vi "order-spectrum-flexlogger-hold-test.vi"(8 "error in (no error)":errorcluster) -> (0 "error out":errorcluster, 1 "Plot Waveform Count":i32[](array[numeric]), 2 "Plot Values":dbl[][][](array[numeric]), 3 "Log Values":dbl[][](array[numeric]), 4 "Log Waveform Count":i32[](array[numeric]))   [LabVIEW 2026]
doc: "Hold/reset unit test for OrderSpectrumToFlexLogger.vi: calls it 5 times with (0) reset + spectrum A, (1) empty magnitude, (2) empty array, (3) spectrum B, (4) reset + empty array. Returns numeric arrays only."
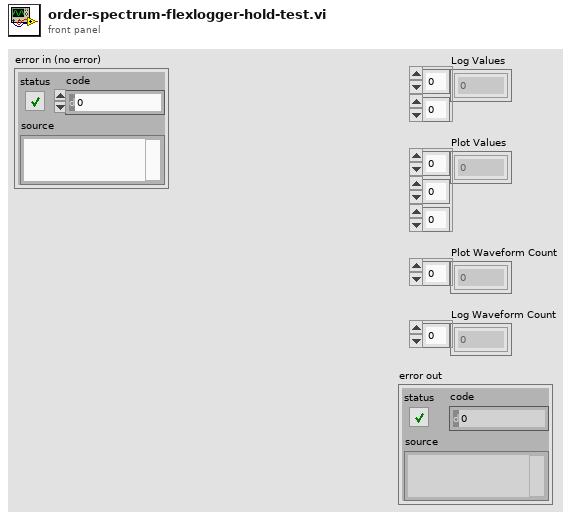
[diagram p1: front panel]
types:
  T1 = cluster{"channels":i32, "plot points per block":i32, "plot in dB? (F)":bool, "window ENBW (bins)":dbl}
  T2 = cluster{"spectra":cluster{"order 0":dbl, "delta order":dbl, "magnitude":dbl[]}[], "reset":bool}[]
  T3 = cluster{"order 0":dbl, "delta order":dbl, "magnitude":dbl[]}[]
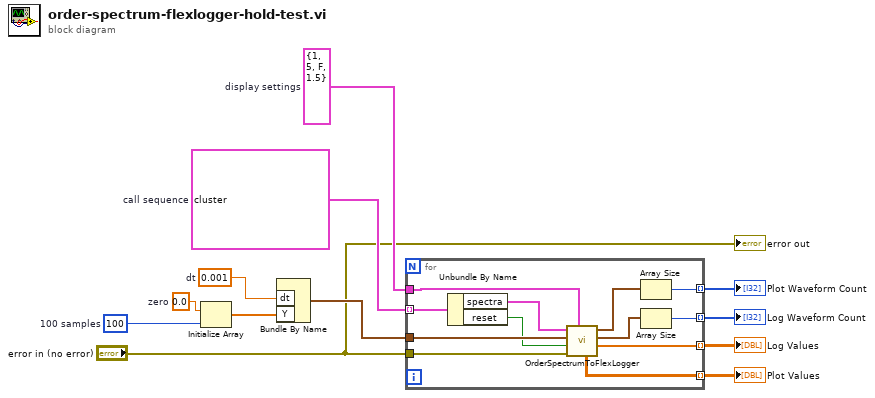
[diagram p0: block diagram]
diagram:
  w6 = T1 {"channels"=1, "plot points per block"=5, "plot in dB? (F)"=FALSE, "window ENBW (bins)"=1.5}  # display settings
  w10 = 0.001  # dt
  w11 = 100  # 100 samples
  w12 = 0.0  # zero
  w8 = T2 [{"spectra"=[{"order 0"=1.0, "delta order"=0.5, "magnitude"=[0.01, 0.04, 0.0025]}], "reset"=TRUE}, {"spectra"=[{"order 0"=1.0, "delta order"=0.5, "magnitude"=[]}], "reset"=FALSE}, {"spectra"=[], "reset"=FALSE}, {"spectra"=[{"order 0"=2.0, "delta order"=0.25, "magnitude"=[0.09, 0.01]}], "reset"=FALSE}, {"spectra"=[], "reset"=TRUE}]  # call sequence
  n1 = Initialize Array(w12, w11) -> (w9:dbl[])
  n2 = Bundle By Name("dt"=w10, "Y"=w9) -> (w7:waveform(dbl))  [unwired: 1 in]
  n3 = for {
    tunnel: w8 -> [w24] mode=indexing
    tunnel: w7 -> [w22]
    tunnel: w6 -> [w19]
    tunnel: "error in (no error)" -> [w20]
    tunnel: [w16] -> w5 mode=indexing
    tunnel: [w15] -> w4 mode=indexing
    tunnel: [w14] -> w3 mode=indexing
    tunnel: [w13] -> w2 mode=indexing
    n4 = Unbundle By Name(w24) -> ("spectra"=w23:T3, "reset"=w21:bool)
    n5 = call "OrderSpectrumToFlexLogger.vi"("Spectrum Display Settings"=w19, "error in (no error)"=w20, "reset? (F)"=w21, "Timing Reference"=w22, "order power spectra"=w23) -> ("Log Values"=w16:dbl[], "Log Waveforms"=w17:waveform(dbl)[], "Plot Waveforms"=w18:waveform(dbl)[], "Plot Values"=w15:dbl[][])  [unwired: 2 in, 1 out]
    n6 = Array Size(array=w18) -> (size(s)=w14:i32)
    n7 = Array Size(array=w17) -> (size(s)=w13:i32)
  }
  "Log Values" <- w5
  "Plot Values" <- w4
  "Plot Waveform Count" <- w3
  "Log Waveform Count" <- w2
  "error out" <- "error in (no error)"
